vi "text_to_speech.vi"() -> ()   [LabVIEW 2018]
uses:
  System.Speech
panel:
  in  "gender":i32(ring) items=["NotSet", "Male", "Female", "Neutral"]
  in  "textToSpeak":string
  # "TEXT TO SPEECH"
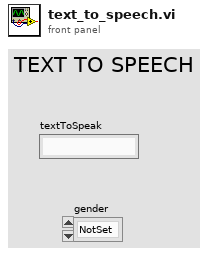
[diagram p1: front panel]
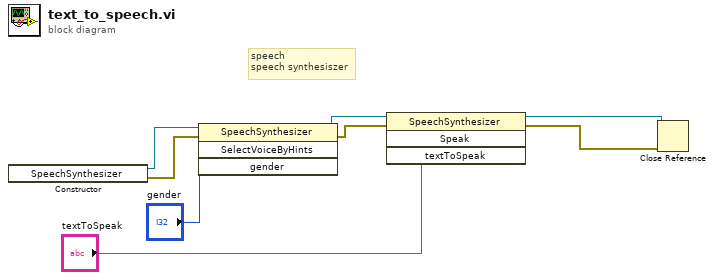
[diagram p0: block diagram]
diagram:
  # "speech\nspeech synthesiszer"
  n1 = constructor class="SpeechSynthesizer"() -> (reference out=w5:refnum<k24>, error out=w4:errorcluster)  [unwired: 3 in, 1 out]
  n2 = invoke class="SpeechSynthesizer" method="SelectVoiceByHints"(reference=w5, error in=w4, "gender"="gender") -> (reference out=w1:refnum<k24>, error out=w3:errorcluster)  [unwired: 1 in, 2 out]
  n3 = invoke class="SpeechSynthesizer" method="Speak"(reference=w1, error in=w3, "textToSpeak"="textToSpeak") -> (reference out=w8:refnum<k24>, error out=w7:errorcluster)  [unwired: 1 in, 2 out]
  n4 = Close Reference(reference=w8, error in (no error)=w7) -> ()  [unwired: 1 out]
